vi "thermal_optical_capture_21.vi"() -> ()   [LabVIEW 2025]
uses:
  <vilib>/vision/driver/NI_Vision_Acquisition_Software.lvlib
  <resource>/objmgr/imaqdx.rc
panel:
  in  "Camera Name":refnum<k21> caption="IMAQdx Session"
  out "error out":errorcluster
  out "max value":u16
  out "Image Pixels (U16)":u16[][](array[numeric])
  out "Image Preview":T1(plugin-control)
  out "FPS":u32
  in  "milliseconds to wait":u32=100
  out "Thermal Preview":T1(plugin-control)
  in  "Stop Preview":bool
  in  "STOP ACQUISITION":bool
  in  "Focus":dbl(slide) scale=0.0..100.0
  out "Thermal Frame Out":string
  in  "Output Folder":path
  in  "thermal capture interval (s)":dbl
  in  "Flag Button":bool
  in  "Stop & Save":bool
  in  "Record":bool
  # "Instructions:\n1) Make sure terminal is closed (from previous sessions)\n2) Inputs: Select camera, data folder path, & milliseconds to wait (~100)\n3) Run VI. (Optical images will begin writing, disregard.)\n4) Wait until terminal gives \"thermal camera calibrated and data reliable\" message\n5) Press Thermal Record \"Start\", both thermal & optical will write files with common timestamps"
  # "Thermal Record"
  # "(Enter \"28\")"
  # "(applies to thermal)"
  # "^ append to base data folder \"...\\raw\\test_n\" for nth recording"
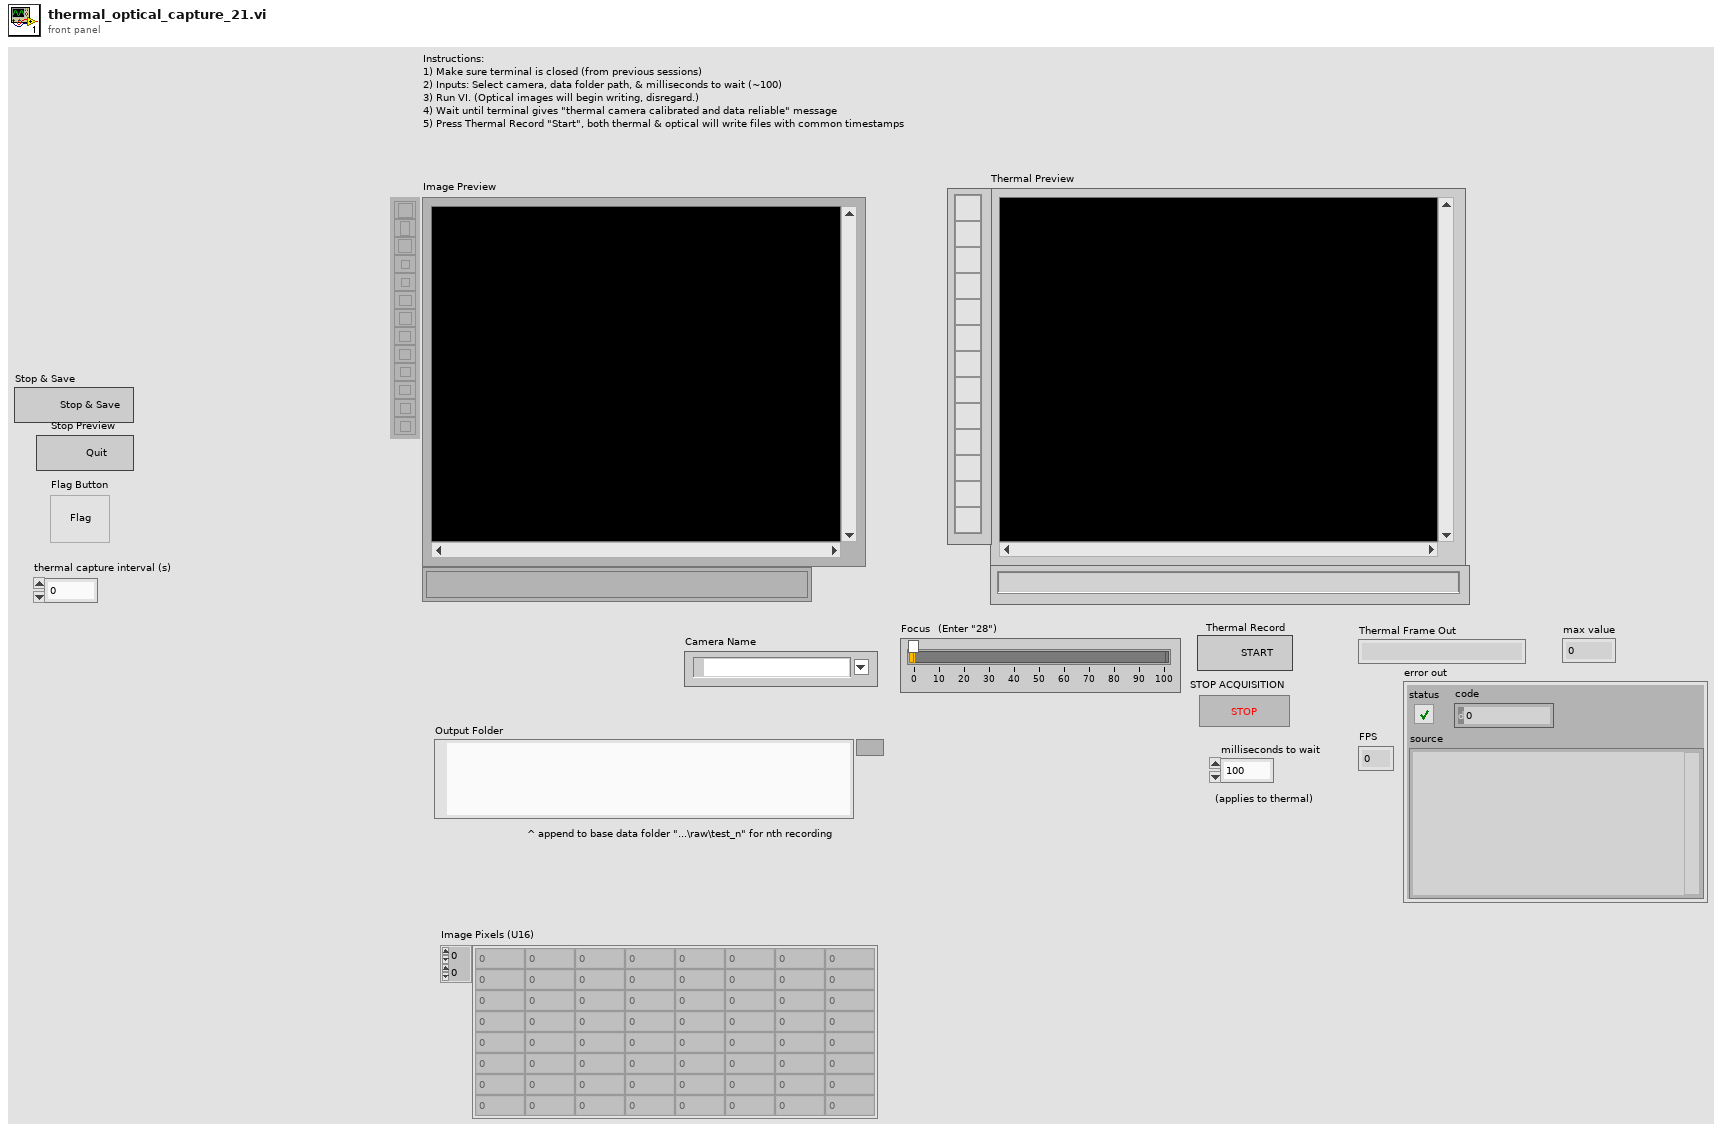
[diagram p1: front panel]
types:
  T1 = typedef "IMAQ Image.ctl" = refnum<image>
  T2 = enum16{"open", "replace", "create", "open or create", "replace or create", "replace or create with confirmation"}
  T3 = enum16{"big-endian, network order", "native, host order", "little-endian"}
  T4 = typedef "Image Type" = u32
  T5 = typedef "IMAQdx.ctl" = refnum<k21>
  T6 = enum16{"Standard", "Buffered", "CRLF", "Immediate"}
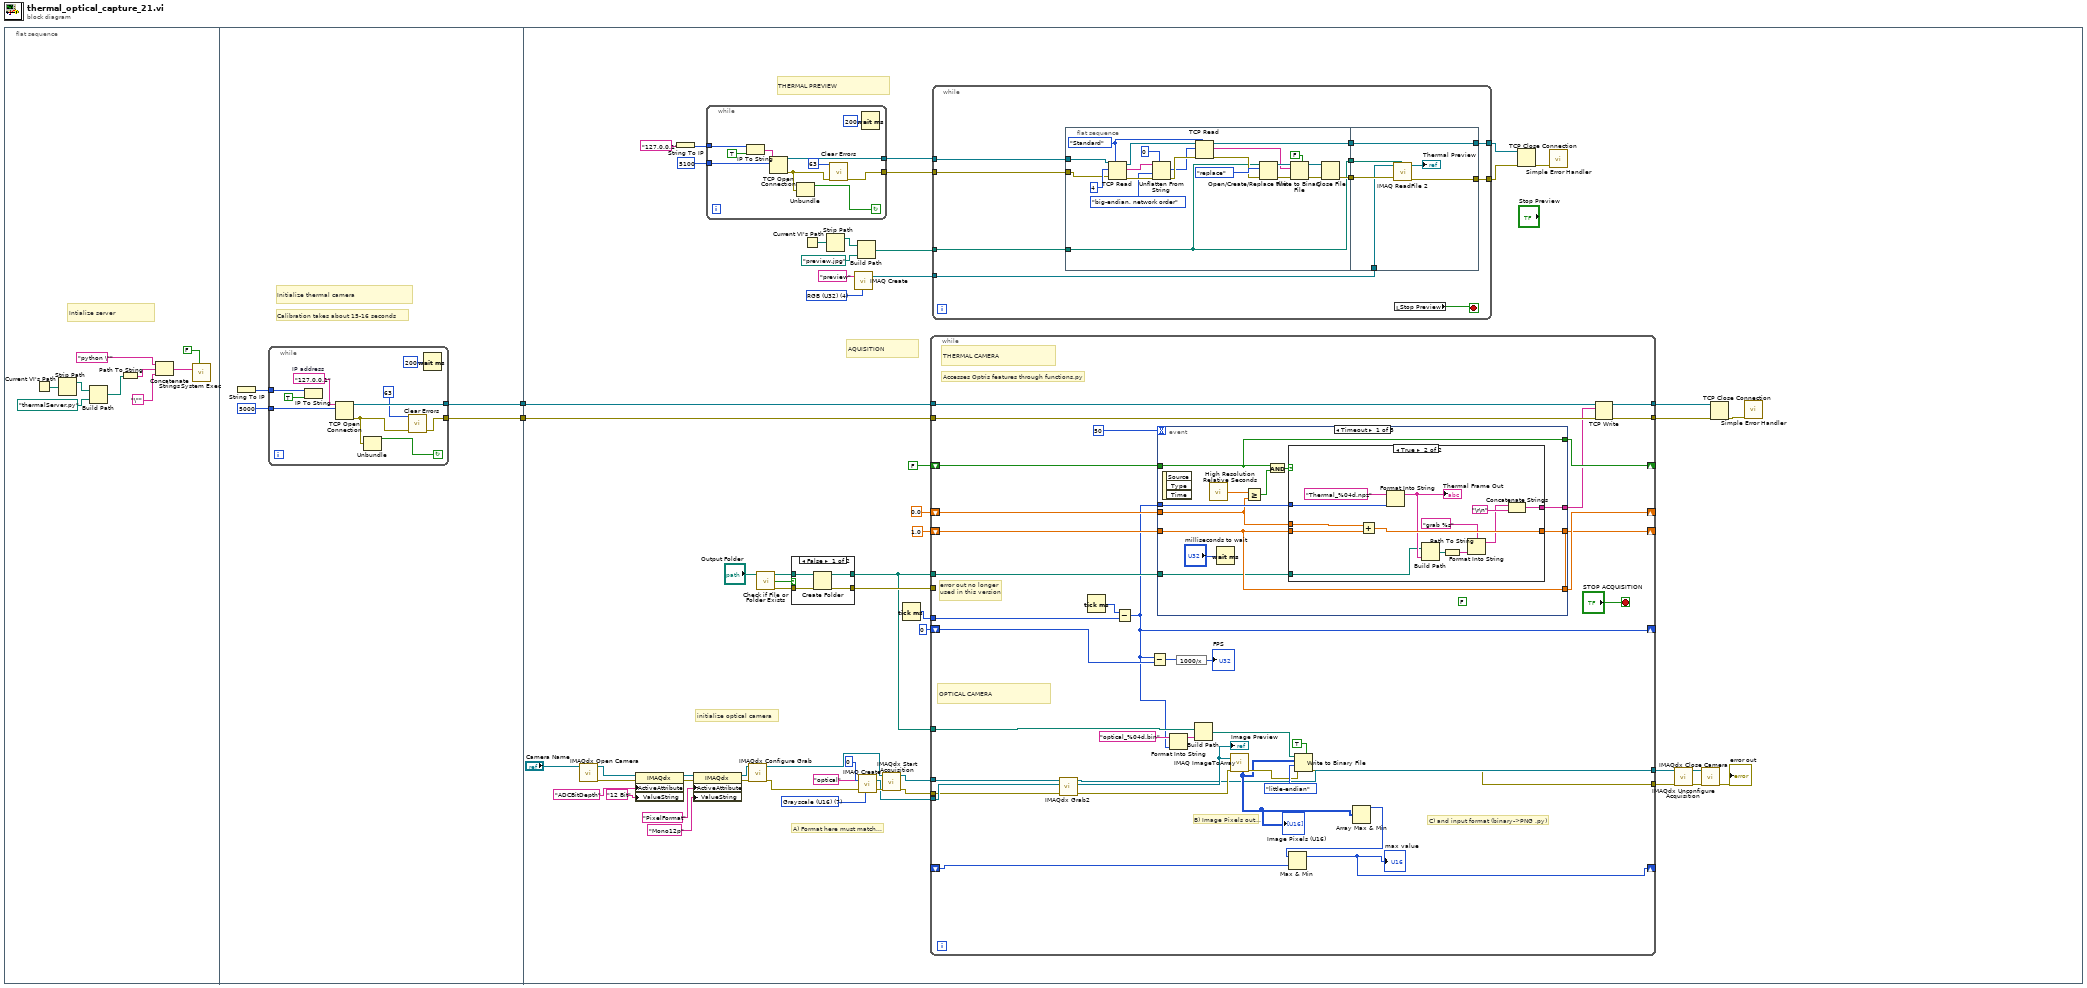
[diagram p0: block diagram]
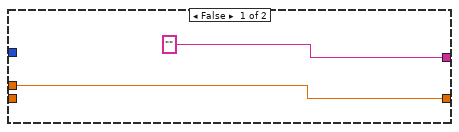
[diagram p3: hidden frame]
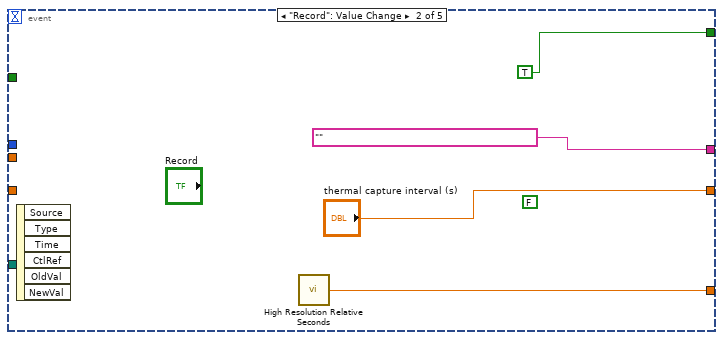
[diagram p4: hidden frame]
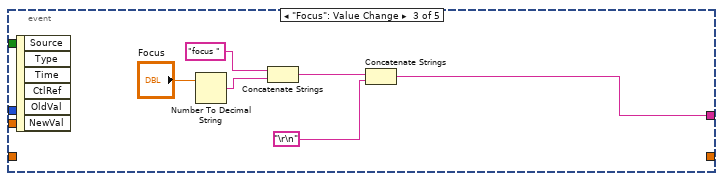
[diagram p5: hidden frame]
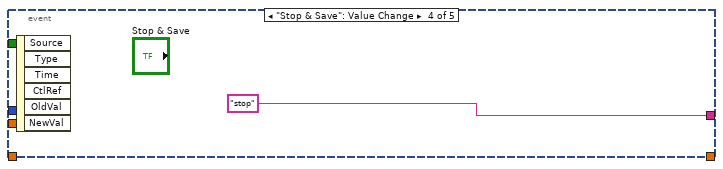
[diagram p6: hidden frame]
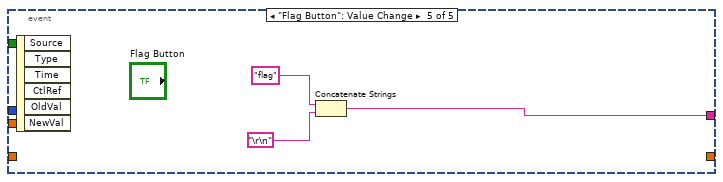
[diagram p7: hidden frame]
diagram:
  n1 = flat-sequence {
    tunnel: [w13] -> w2
    tunnel: [w12] -> w1
    tunnel: w1 -> [w77]
    tunnel: w2 -> [w76]
    frame #0 {
      # "Intialize server"
      n2 = Current VI's Path() -> (path=w6:path)
      n3 = Strip Path(path=w6) -> (stripped path=w7:path)  [unwired: 1 out]
      n4 = Build Path(base path=w7, name or relative path=path "thermalServer.py") -> (appended path=w4:path)
      n5 = Path To String(path=w4) -> (string=w10:string)
      n6 = Concatenate Strings("python \"" ("string"), w10, "\"" ("string")) -> (w9:string)
      n7 = call <vilib>:"System Exec.vi"("wait until completion? (T)"=FALSE, "command line"=w9) -> ()  [unwired: 6 in, 4 out]
    }
    frame #1 {
      # "Initialize thermal camera"
      # "Calibration takes about 15-16 seconds"
      n8 = String To IP() -> (0:w15:u32)  [unwired: 1 in]
      n9 = while {
        tunnel: [w20] -> w13
        tunnel: [w25] -> w12
        tunnel: w15 -> [w24]
        tunnel: u16 5000 ("remote port or service name") -> [w22]
        stop <- w17 continue-if-true
        w16 = "127.0.0.1"  # IP address
        n10 = IP To String(1:TRUE ("dot notation? (F)"), 2:w24) -> ()  [unwired: 1 out]
        n11 = TCP Open Connection(address=w16, remote port or service name=w22) -> (connection ID=w25:refnum<k5>, error out=w21:errorcluster)  [unwired: 3 in]
        n12 = Unbundle(w21) -> ("status"=w17:bool)  [unwired: 2 out]
        n13 = call <vilib>:"Clear Errors.vi"("error in (no error)"=w21, "specific error code to clear (0: all)"=63) -> ("error out"=w20:errorcluster)  [unwired: 4 in, 1 out]
        n14 = Wait (ms)(milliseconds to wait=u32 200) -> ()  [unwired: 1 out]
      }
    }
    frame #2 {
      w44 = T4 7 items=["Grayscale (U8)", "Grayscale (I16)", "Grayscale (SGL)", "Complex (CSG)", "RGB (U32)", "HSL (U32)", "RGB (U64)", "Grayscale (U16)"] ("Image Type")
      w65 = T4 4 items=["Grayscale (U8)", "Grayscale (I16)", "Grayscale (SGL)", "Complex (CSG)", "RGB (U32)", "HSL (U32)", "RGB (U64)", "Grayscale (U16)"] ("Image Type")
      # "A) Format here must match..."
      # "initialize optical camera"
      # "THERMAL PREVIEW"
      # "AQUISITION"
      n15 = call <vilib>:"IMAQdx Open Camera.vi"("Session In"="Camera Name") -> ("error out"=w41:errorcluster, "Session Out"=w42:T5)  [unwired: 9 in]
      n16 = property class="IMAQdx"(reference=w42, error in=w41, "ActiveAttribute"="ADCBitDepth", "ValueString"="12 Bit") -> (reference out=w34:T5, error out=w32:errorcluster)
      n17 = String To IP(1:"127.0.0.1" ("name")) -> (0:w64:u32)
      n18 = property class="IMAQdx"(reference=w34, error in=w32, "ActiveAttribute"="PixelFormat", "ValueString"="Mono12p" ("ActiveAttribute")) -> (reference out=w33:T5, error out=w31:errorcluster)
      n19 = while {
        tunnel: w64 -> [w96]
        tunnel: [w90] -> w63
        tunnel: [w94] -> w62
        tunnel: u16 5100 ("remote port or service name") -> [w92]
        stop <- w87 continue-if-true
        n20 = IP To String(1:TRUE ("dot notation? (F)"), 2:w96) -> (0:w95:string)
        n21 = TCP Open Connection(address=w95, remote port or service name=w92) -> (connection ID=w94:refnum<k5>, error out=w91:errorcluster)  [unwired: 3 in]
        n22 = Unbundle(w91) -> ("status"=w87:bool)  [unwired: 2 out]
        n23 = call <vilib>:"Clear Errors.vi"("error in (no error)"=w91, "specific error code to clear (0: all)"=63) -> ("error out"=w90:errorcluster)  [unwired: 4 in, 1 out]
        n24 = Wait (ms)(milliseconds to wait=u32 200) -> ()  [unwired: 1 out]
      }
      n25 = call <vilib>:"IMAQdx Configure Grab.vi"("error in"=w31, "Session In"=w33) -> ("error out"=w38:errorcluster, "Session Out"=w37:T5)  [unwired: 8 in]
      n26 = call <vilib>:"Check if File or Folder Exists.vi"("path"="Output Folder") -> ("error out"=w57:errorcluster, "file or folder exists?"=w59:bool)  [unwired: 8 in, 1 out]
      n27 = case shown="False" w59 {
        tunnel: "Output Folder" -> [w84 w86]
        tunnel: [w83 w86] -> w51
        tunnel: w57 -> [w82 w85]
        tunnel: [w81 w85] -> w56
        frame False {
          n28 = Create Folder(path (use dialog)=w84, error in=w82) -> (created path=w83:path, error out=w81:errorcluster)  [unwired: 1 in, 1 out]
        }
        frame True {
        }
      }
      n29 = Current VI's Path() -> (path=w70:path)
      n30 = Strip Path(path=w70) -> (stripped path=w71:path)  [unwired: 1 out]
      n31 = call "IMAQ Create"("Image Name"="preview", "Image Type"=w65) -> ("New Image"=w68:T1)  [unwired: 3 in, 1 out]
      n32 = Build Path(base path=w71, name or relative path=path "preview.jpg") -> (appended path=w69:path)
      n33 = call "IMAQ Create"("Border Size"=0, "Image Name"="optical", "Image Type"=w44, "error in (no error)"=w38) -> ("New Image"=w27:T1, "error out"=w39:errorcluster)  [unwired: 1 in]
      n34 = call <vilib>:"IMAQdx Start Acquisition.vi"("error in"=w39, "Session In"=w37) -> ("error out"=w26:errorcluster, "Session Out"=w28:T5)  [unwired: 8 in]
      n35 = Tick Count (ms)() -> (millisecond timer value=w72:u32)
      n36 = while {
        tunnel: [w172] -> w78
        tunnel: [w171] -> w79
        tunnel: w77 -> [w170]
        tunnel: w76 -> [w169]
        shift-right: [w168] -> _
        shift-left: 0.0 -> [w165]
        shift-right: [w166] -> _
        shift-left: 1.0 -> [w163]
        shift-right: [w167] -> _
        shift-left: FALSE -> [w164]
        tunnel: w72 -> [w156]
        shift-right: [w138] -> _
        shift-left: u32 0 -> [w157]
        tunnel: w51 -> [w158]
        tunnel: w56 -> [_]
        tunnel: w51 -> [w143]
        tunnel: [w142] -> w47
        tunnel: [w141] -> w46
        shift-right: [w139] -> _
        shift-left: _ -> [w140]
        tunnel: w28 -> [w137]
        tunnel: w27 -> [w136]
        tunnel: w26 -> [w135]
        stop <- "STOP ACQUISITION" stop-if-true
        # "C) and input format (binary->PNG .py)"
        # "B) Image Pixels out..."
        # "OPTICAL CAMERA"
        # "error out no longer used in this version"
        # "THERMAL CAMERA"
        # "Accesses Optris features through functions.py"
        n37 = call <vilib>:"IMAQdx Grab2.vi"("error in"=w135, "Image In"=w136, "Session In"=w137) -> ("error out"=w147:errorcluster, "Image Out"=w148:T1, "Session Out"=w142:T5)  [unwired: 5 in, 1 out]
        "Image Preview" <- w148
        n38 = Tick Count (ms)() -> (millisecond timer value=w159:u32)
        n39 = Subtract(x=w159, y=w156) -> (x-y=w138:u32)
        n40 = Subtract(x=w138, y=w157) -> (x-y=w155:u32)
        n41 = event shown="[0] Timeout" {
          selector: _ -> [_ _ _ _ _]
          dyn-events: _ -> [_ _ _ _ _]
          timeout: 50 -> [_ _ _ _ _]
          tunnel: [w179 "" w203 "stop" w212] -> w160
          tunnel: w138 -> [w180 _ _ _ _]
          tunnel: [w177 w202 _ _ _] -> w168
          tunnel: [w175 TRUE _ _ _] -> w167
          tunnel: [w176 "thermal capture interval (s)" _ _ _] -> w166
          tunnel: w165 -> [w178 _ _ _ _]
          tunnel: w164 -> [w175 _ _ _ _]
          tunnel: w163 -> [w176 _ _ _ _]
          tunnel: w158 -> [w174 _ _ _ _]
          event Timeout {
            (unwired) FALSE
            n42 = event-data() -> ()  [unwired: 1 in, 3 out]
            n43 = call <vilib>:"High Resolution Relative Seconds.vi"() -> ("relative seconds"=w183:dbl)
            n44 = Wait (ms)(milliseconds to wait="milliseconds to wait") -> ()  [unwired: 1 out]
            n45 = Greater Or Equal?(x=w183, y=w178) -> (x >= y?=w182:bool)
            n46 = And(x=w175, y=w182) -> (x .and. y?=w181:bool)
            n47 = case shown="True" w181 {
              tunnel: w180 -> [_ w196]
              tunnel: ["" w197] -> w179
              tunnel: w178 -> [w184 w195]
              tunnel: w176 -> [_ w194]
              tunnel: [w184 w193] -> w177
              tunnel: w174 -> [_ w186]
              frame False {
              }
              frame True {
                n48 = Add(x=w195, y=w194) -> (x+y=w193:dbl)
                n49 = Format Into String(format string="Thermal_%04d.npz", w196) -> (resulting string=w187:string)  [unwired: 2 in, 1 out]
                "Thermal Frame Out" <- w187
                n50 = Build Path(base path=w186, name or relative path=w187) -> (appended path=w191:path)
                n51 = Path To String(path=w191) -> (string=w189:string)
                n52 = Format Into String(format string="grab %s", w189) -> (resulting string=w188:string)  [unwired: 2 in, 1 out]
                n53 = Concatenate Strings(w188, "\r\n") -> (w197:string)
              }
            }
          }
          event "Record": Value Change {
            (unwired) FALSE
            n54 = event-data() -> ()  [unwired: 1 in, 6 out]
            n55 = call <vilib>:"High Resolution Relative Seconds.vi"() -> ("relative seconds"=w202:dbl)
          }
          event "Focus": Value Change {
            n56 = event-data() -> ()  [unwired: 1 in, 6 out]
            n57 = Number To Decimal String(number="Focus") -> (decimal integer string=w208:string)  [unwired: 1 in]
            n58 = Concatenate Strings("focus ", w208) -> (w205:string)
            n59 = Concatenate Strings(w205, "\r\n") -> (w203:string)
          }
          event "Stop & Save": Value Change {
            n60 = event-data() -> ()  [unwired: 1 in, 6 out]
          }
          event "Flag Button": Value Change {
            n61 = event-data() -> ()  [unwired: 1 in, 6 out]
            n62 = Concatenate Strings("flag", "\r\n") -> (w212:string)
          }
        }
        n63 = Format Into String(format string="optical_%04d.bin", w138) -> (resulting string=w153:string)  [unwired: 2 in, 1 out]
        n64 = expression code="1000/x"(w155) -> (→"FPS":u32)
        n65 = Build Path(base path=w143, name or relative path=w153) -> (appended path=w151:path)
        n66 = call "IMAQ ImageToArray"("error in (no error)"=w147, "Image"=w148) -> ("Image Pixels (U16)"=w145:u16[][], "error out"=w146:errorcluster)  [unwired: 2 in, 3 out]
        "Image Pixels (U16)" <- w145
        n67 = Write to Binary File(file (use dialog)=w151, data=w145, error in=w146, 5:TRUE, 9:T3."little-endian" ("byte order (0:big-endian, network order)")) -> (error out=w141:errorcluster)  [unwired: 1 in, 2 out]
        n68 = Array Max & Min(array=w145) -> (max value=w144:u16)  [unwired: 3 out]
        n69 = Max & Min(x=w144, y=w140) -> (max(x,y)=w139:u16)  [unwired: 1 out]
        "max value" <- w139
        n70 = TCP Write(connection ID=w170, data in=w160, error in (no error)=w169) -> (connection ID out=w171:refnum<k5>, error out=w172:errorcluster)  [unwired: 1 in, 1 out]
      }
      n71 = while {
        tunnel: w68 -> [w101]
        tunnel: [w102] -> w54
        tunnel: [w106] -> w53
        tunnel: w69 -> [w104]
        tunnel: w63 -> [w99]
        tunnel: w62 -> [w98]
        stop <- w97 stop-if-true
        n72 = flat-sequence {
          tunnel: w104 -> [w110]
          tunnel: [w112] -> w105
          tunnel: [w111] -> w103
          tunnel: [w110] -> w100
          tunnel: w99 -> [w108]
          tunnel: w98 -> [w107]
          tunnel: [w134] -> w106
          tunnel: w105 -> [w134]
          tunnel: w103 -> [w133]
          tunnel: [w132] -> w102
          tunnel: w101 -> [w131]
          tunnel: w100 -> [w130]
          frame #0 {
            w121 = T6."Standard" ("mode (standard)")
            n73 = TCP Read(connection ID=w107, bytes to read=4, error in (no error)=w108, 7:w121) -> (connection ID out=w124:refnum<k5>, data out=w109:string, error out=w127:errorcluster)  [unwired: 1 in]
            n74 = Unflatten From String(type=0, binary string=w109, byte order (0:big-endian, network order)=T3."big-endian, network order", error in (no error)=w127) -> (value=w122:i32, error out=w123:errorcluster)  [unwired: 1 in, 1 out]
            n75 = TCP Read(connection ID=w124, bytes to read=w122, error in (no error)=w123, 7:w121) -> (connection ID out=w112:refnum<k5>, data out=w117:string, error out=w119:errorcluster)  [unwired: 1 in]
            n76 = Open/Create/Replace File(file path (use dialog)=w110, error in=w119, operation (0:open)=T2."replace") -> (refnum out=w118:refnum<file>, error out=w115:errorcluster)  [unwired: 3 in, 1 out]
            n77 = Write to Binary File(file (use dialog)=w118, data=w117, error in=w115, 5:FALSE ("prepend array or string size? (T)")) -> (refnum out=w113:refnum<file>, error out=w114:errorcluster)  [unwired: 2 in, 1 out]
            n78 = Close File(refnum=w113, error in=w114) -> (error out=w111:errorcluster)  [unwired: 1 out]
          }
          frame #1 {
            n79 = call "IMAQ ReadFile 2"("File Path"=w130, "error in (no error)"=w133, "Image"=w131) -> ("error out"=w132:errorcluster, "Image Out"=→"Thermal Preview":T1)  [unwired: 4 in, 3 out]
          }
        }
        n80 = local read "Stop Preview"() -> (w97:bool)
      }
      n81 = TCP Close Connection(connection ID=w53, error in (no error)=w54) -> (error out=w55:errorcluster)  [unwired: 1 in, 1 out]
      n82 = call <vilib>:"Simple Error Handler.vi"("error in (no error)"=w55) -> ()  [unwired: 4 in, 5 out]
      n83 = call <vilib>:"IMAQdx Unconfigure Acquisition.vi"("error in"=w46, "Session In"=w47) -> ("error out"=w48:errorcluster, "Session Out"=w49:T5)  [unwired: 8 in]
      n84 = call <vilib>:"IMAQdx Close Camera.vi"("error in"=w48, "Session In"=w49) -> ("error out"=→"error out":errorcluster)  [unwired: 9 in]
      n85 = TCP Close Connection(connection ID=w79, error in (no error)=w78) -> (error out=w80:errorcluster)  [unwired: 1 in, 1 out]
      n86 = call <vilib>:"Simple Error Handler.vi"("error in (no error)"=w80) -> ()  [unwired: 4 in, 5 out]
    }
  }
